vi "Render_UI_Task.vi"(8 "error in (no error)":errorcluster={"status"=FALSE, "code"=0, "source"="\"\""}, 9 "Condition Met":bool=TRUE, 10 "Measured Pressure":dbl=100.0, 11 "Step Index":i32=1) -> (0 "error out":errorcluster, 2 "Tolerance LED":bool, 3 "UI String":string)   [LabVIEW 2026]
doc: "Worker task that formats live indicators and status message for display."
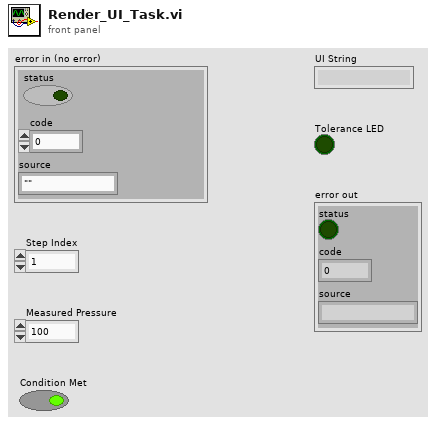
[diagram p1: front panel]
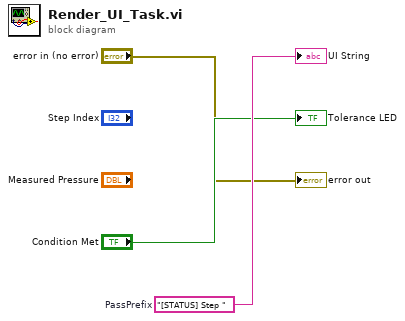
[diagram p0: block diagram]
diagram:
  w3 = "[STATUS] Step "  # PassPrefix
  "UI String" <- w3
  "Tolerance LED" <- "Condition Met"
  "error out" <- "error in (no error)"
